vi "ZM-CP-FL-buildPath.vi"(8 "error in (no error)":errorcluster, 10 "type_name":string, 11 "folder":path) -> (0 "error out":errorcluster, 3 "file":path)   [LabVIEW 2020, in "ZM-CP-FL-file_logger.lvlib" / "ZM-CP-FL-file_logger.lvclass"]
doc: "Builds the JSON Lines file path of one package type: <folder>/<type_name>.jsonl, one file per package type. No node here raises an error."
uses:
  ZM-CP-FL-file_logger.lvclass
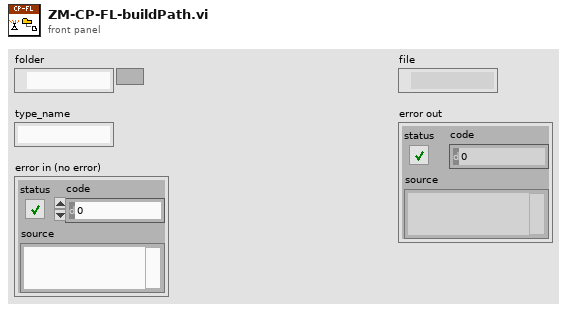
[diagram p1: front panel]
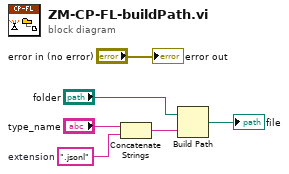
[diagram p0: block diagram]
diagram:
  w5 = ".jsonl"  # extension
  n1 = Concatenate Strings("type_name", w5) -> (w3:string)
  n2 = Build Path(base path="folder", name or relative path=w3) -> (appended path=→"file":path)
  "error out" <- "error in (no error)"
